vi "VIH UI - Undo Focused Control - Mouse Click.vi"(8 "error in":errorcluster, 11 "VI Refnum":refnum<vi>) -> (0 "error out":errorcluster, 3 "dup VI Refnum":refnum<vi>)   [LabVIEW 2014]
doc: "::: VI Helpeks :::\nCopyright (c) 2000-2026 Konstantin Shifershteyn. All rights reserved."
panel:
  # "VI Helpeks\nCopyright (c) 2012-2026 Konstantin Shifershteyn"
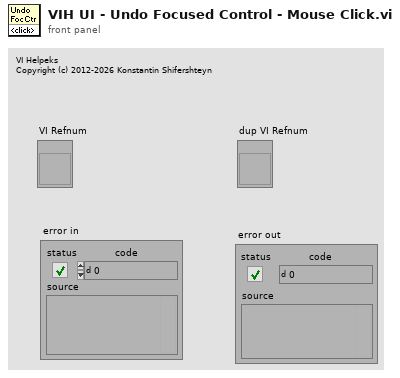
[diagram p1: front panel]
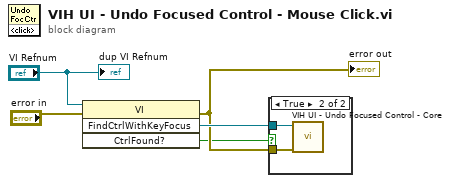
[diagram p0: block diagram]
diagram:
  n1 = invoke class="VI" method="FindCtrlWithKeyFocus"(reference="VI Refnum", error in="error in") -> (error out=w3:errorcluster, "FindCtrlWithKeyFocus"=w5:refnum<vi>, "CtrlFound?"=w1:bool)  [unwired: 2 in, 1 out]
  "error out" <- w3
  n2 = case shown="True" w1 {
    tunnel: w5 -> [_ w7]
    tunnel: w3 -> [_ w6]
    frame False {
    }
    frame True {
      n3 = call "VIH UI - Undo Focused Control - Core.vi"("error in"=w6, "Ctl Refnum"=w7) -> ()  [unwired: 7 in, 3 out]
    }
  }
  "dup VI Refnum" <- "VI Refnum"
